vi "!GviewerMain.vi"() -> ()   [LabVIEW 2020, in "Sgraph_lib_V1.lvlib" / "Gviewer.lvclass"]
doc: "Main Graph Viewer.\nSeveral instances of this viewer can run simultaneously."
uses:
  Gviewer.lvclass
  controls/Typedef_Live.ctl
  Gserver/controls/Typedef_Gviewer-Query.ctl
  Gserver/controls/Typedef_QueryType.ctl
  controls/KeyPress.ctl
  <vilib>/event_ctls.llb/eventvkey.ctl
  Gviewer.lvclass/Gviewer.ctl
  FAMM/controls/FAMM_reply_datagram.ctl
  FAMM/controls/FAMM_reply_WAQdata.ctl
  FAMM/controls/FAMM_reply_EAQdata.ctl
  FAMM/controls/FAMM_reply_PAQdata.ctl
  controls/EditTagOneTag.ctl
  controls/Typedef_SelProperties.ctl
  controls/Typedef_LineType.ctl
  controls/Typedef_PresetSave.ctl
  controls/ToolBarAppearance.ctl
  controls/Typedef_Gserver-Replies.ctl
  controls/Typedef_ServerActions.ctl
  Common/controls/ToolTypeEnum.ctl
  Gserver/Gserver.lvclass
  FAMM/FAMM.lvclass
  Builds/Sgraph_lib_V1.lvlib
panel:
  out "TimeSpanText":string
  out "Key UP":T1 {"Time" format="%<%.3X>T"}
  out "Key DN":T1 {"Time" format="%<%.3X>T"}
  in  "StartupTagList":string[](array[string])
  in  "Gserver-Queue":refnum<queue>
  in  "GviewName":string="Gview-01"
  in  "Live":T3
  out "ToolBar":picture
  out "Graph":cluster{dbl[], "data":dbl[]}[](graph)
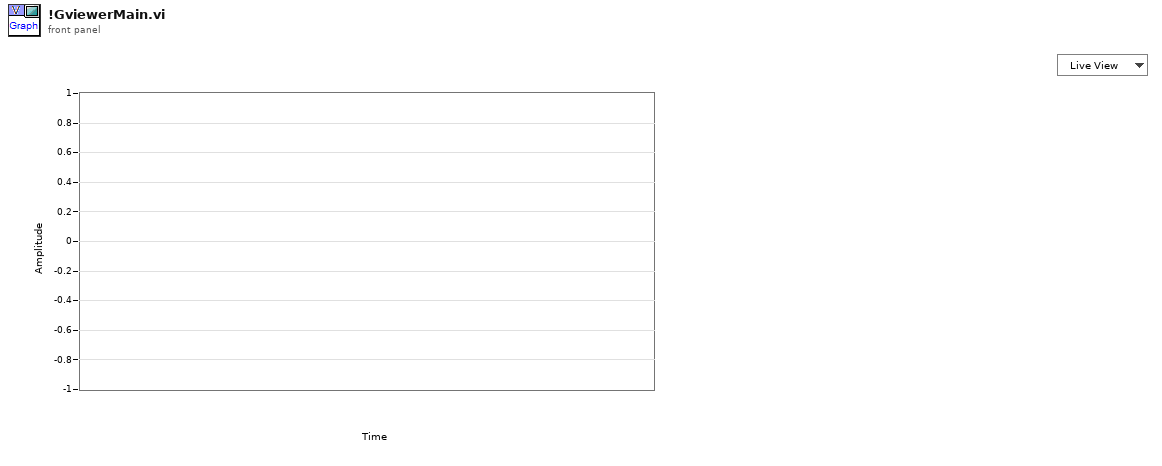
[diagram p1: front panel]
types:
  T1 = typedef "Sgraph_lib_V1.lvlib/Gviewer.lvclass/KeyPress.ctl" = cluster{"Char":i16, "VKey":T2, "Shift":bool, "Ctrl":bool, "Time":timestamp}
  T2 = typedef "eventvkey.ctl" = enum16{"ASCII", "Enter", "Return", "Shift", "Ctrl", "Alt", "Cmd", "Opt", "Caps", "NumLock", "Clear", "Break", "Up", "Down", "Left", "Right", "Insert", "Delete", "Home", "End", "PageUp", "PageDown", "Escape", "Help", "Pause", "ScrollLock", "F1", "F2", "F3", "F4", "F5", "F6", "F7", "F8", "F9", "F10", "F11", "F12", "F13", "F14", "F15", "F16", "F17", "F18", "F19", "F20", "F21", "F22", "F23", "F24", "Play", "VolumeUp", "VolumeDown", "Mute", "Two Byte Char"}
  T3 = typedef "Sgraph_lib_V1.lvlib/Gviewer.lvclass/Typedef_Live.ctl" = enum16{"Live View", "Freeze"}
  T4 = typedef "Sgraph_lib_V1.lvlib/FAMM.lvclass/FAMM_reply_datagram.ctl" = cluster{"GraphName":string, "Time-Start":timestamp, "Time-End":timestamp, "TimeSpan":dbl, "Live":T3, "WAQ_section":T5, "EAQ_section":T6, "PAQ_section":T7, "Layer":i32}
  T5 = typedef "Sgraph_lib_V1.lvlib/FAMM.lvclass/FAMM_reply_WAQdata.ctl" = cluster{"Boolean":bool}
  T6 = typedef "Sgraph_lib_V1.lvlib/FAMM.lvclass/FAMM_reply_EAQdata.ctl" = cluster{"Boolean":bool}
  T7 = typedef "Sgraph_lib_V1.lvlib/FAMM.lvclass/FAMM_reply_PAQdata.ctl" = cluster{"Tags":string[], "time stamp":timestamp[], "DataSection":cluster{"data":dbl[], "max":dbl[], "min":dbl[], "Status":u32[]}[]}
  T8 = typedef "Sgraph_lib_V1.lvlib/Gviewer.lvclass/EditTagOneTag.ctl" = cluster{"TAG":string, "min":dbl, "max":dbl, "Color":u32}
  T9 = typedef "Sgraph_lib_V1.lvlib/Gviewer.lvclass/Typedef_LineType.ctl" = enum16{"num_bare", "num_MinMax_Area", "num_MinMax_Lines", "num_MinMax_Forfor", "num_Max_Area", "num_Max_Line", "num_Max_Forfor", "num_Min_Area", "num_Min_Line", "num_Min_Fosfor", "Boolean_Line_01", "Boolean_Area_01", "Boolean_Fosfor_01", "Boolean_Line_TF", "Boolean_Area_TF", "Boolean_Fosfor_TF", "Boolean_OnOff_Line", "Boolean_OnOff_Area", "Boolean_OnOff_Fosfor", "Boolean_spare", "StringEvent_Line", "StringEvent_TimeLine"}
  T10 = typedef "Sgraph_lib_V1.lvlib/Gviewer.lvclass/Typedef_SelProperties.ctl" = cluster{"Color":u32, "LineType":T9, "max":dbl, "min":dbl}
  T11 = cluster{"EditTagsOpen":bool, "ExitRef":refnum<vi>}
  T12 = typedef "Sgraph_lib_V1.lvlib/Gviewer.lvclass/Typedef_PresetSave.ctl" = cluster{"Save time?":bool, "Presets":T8[], "PresetFilePath":path}
  T13 = typedef "Sgraph_lib_V1.lvlib/Gserver.lvclass/Typedef_QueryType.ctl" = enum16{"Subscribe", "DataRequest", "RequestAllTags", "RequestIniPath", "FAMMstarted", "SetClientOptions", "GviewerUpdate", "OpenNewGraph", "CloseClient", "CloseAllClients", "Close Gserver", "OpenMemoryMap", "MeMapDataRequest", "MeMapDataResponse"}
  T14 = typedef "Sgraph_lib_V1.lvlib/Gviewer.lvclass/ToolBarAppearance.ctl" = enum16{"Bare", "Native", "Gradient"}
  T15 = typedef "Sgraph_lib_V1.lvlib/Typedef_ServerActions.ctl" = enum16{"GraphUpdate", "SendAllTags", "SendIniPath", "SetGeneralOptions", "EditTagsOpen", "EditTagsPresetSave", "EditTagsPresetLoad", "EditTagsClose", "NewTagSelection", "ExitGraph"}
  T16 = typedef "Typedef_Gserver-Replies.ctl" = cluster{"ServerActions":T15, "data":variant, "Source":string, "Time Stamp":timestamp}
  T17 = typedef "Sgraph_lib_V1.lvlib/ToolTypeEnum.ctl" = enum16{"Esc button", "one", "HelpButton", "CursorViewButton", "four", "five", "six", "seven", "eight", "nine", "ten", "eleven", "twelve", "thirteen", "fourteen", "fifteen", "sixteen", "seventeen", "eighteen", "nineteen", "VerticalScroll", "VerticalMove", "TimeScroll", "TimeHandMove", "twentyfour", "twentyfive", "ZoomWindow drag", "ZoomHorDragging", "ZoomVerticalDrag", "twentynine", "LegendMovePoint", "LegendMoveDrag", "Thirtytwo", "ThirtyThree", "ThirtyFour", "ThirgyFive", "ThirtySix", "ThirtySeven", "ThirtyEight", "ThirtyNine", "AddYscalePoint", "AddYscalePlace", "AddYscaleMovePoint", "AddYscaleMoveDrag", "AddYscaleDeletePoint"}
  T18 = typedef "Sgraph_lib_V1.lvlib/Gviewer.lvclass/SettingsGeneral.ctl" = cluster{"MenuBar_active":bool, "ContextMenu_active":bool}
  T19 = typedef "LVPositionTypeDef.ctl" = cluster{"Left":i32, "Top":i32}
  T20 = typedef "LVPoint32TypeDef.ctl" = cluster{"Horizontal":i32, "Vertical":i32}
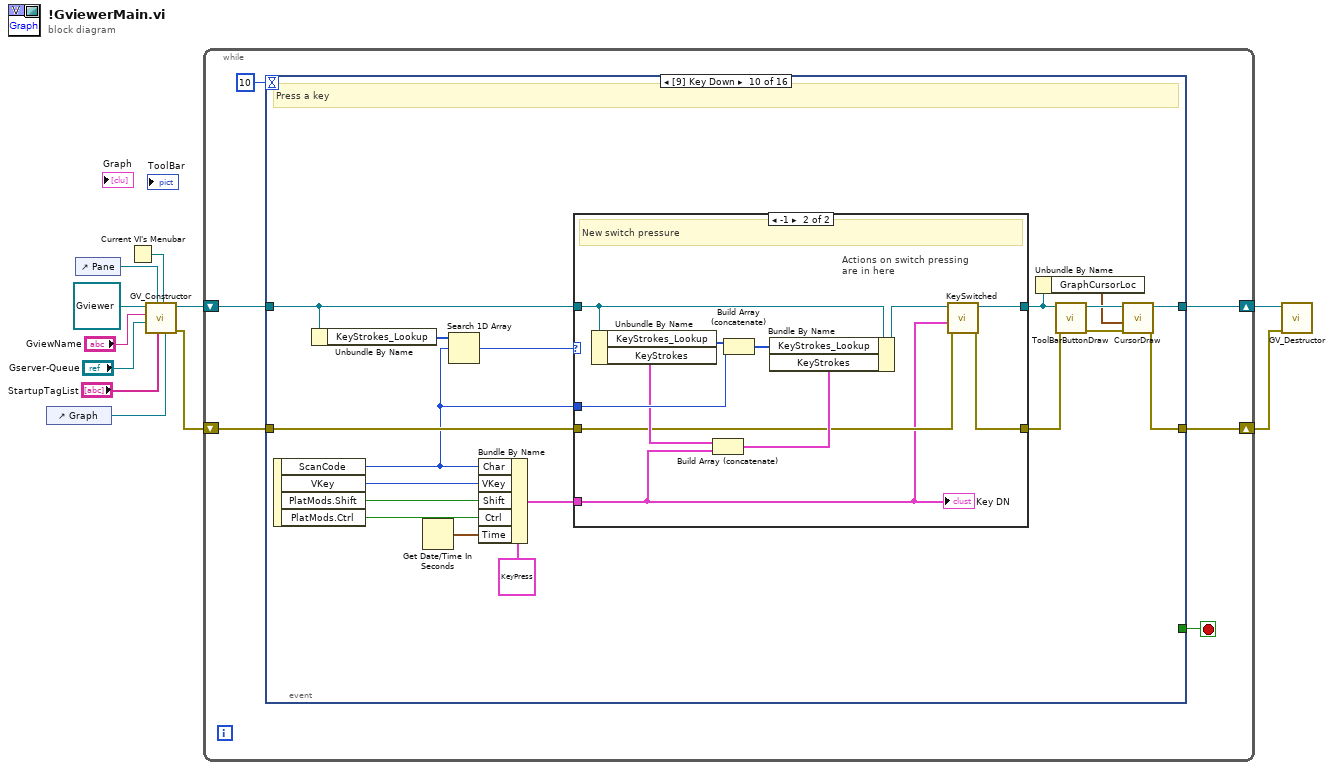
[diagram p0: block diagram]
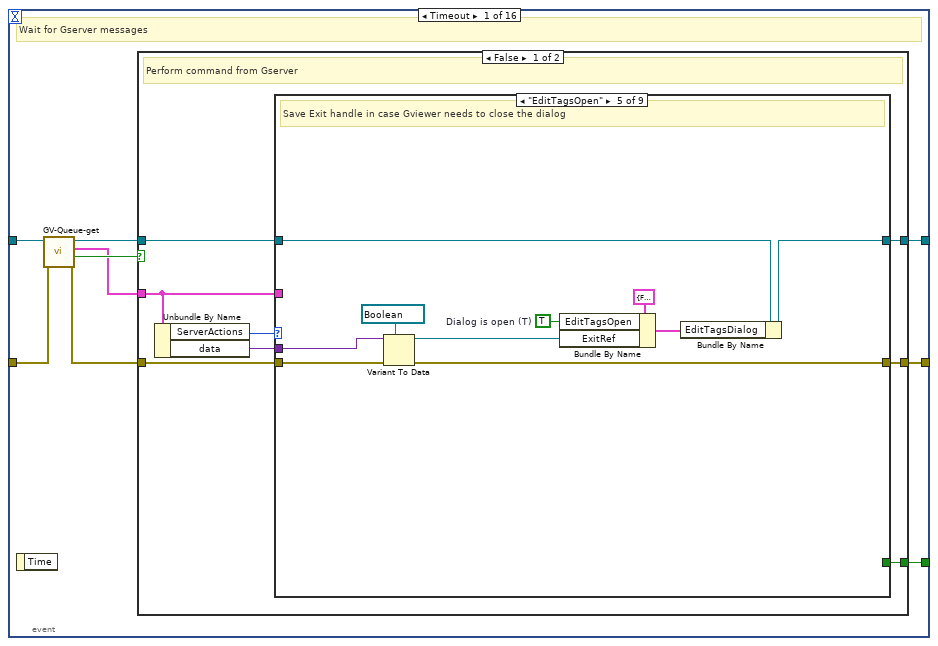
[diagram p2: hidden frame]
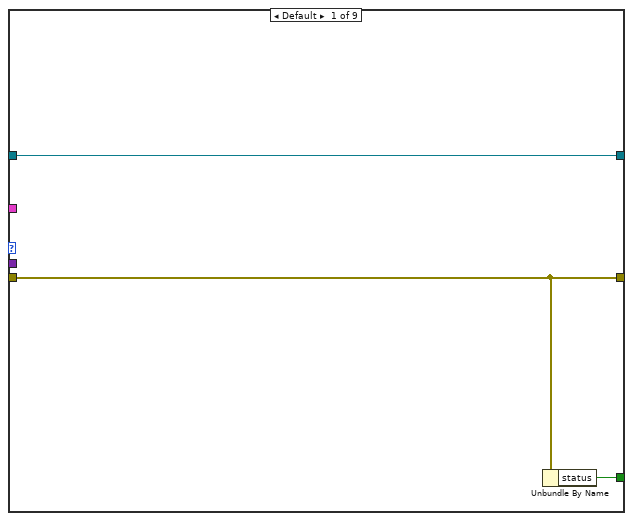
[diagram p3: hidden frame]
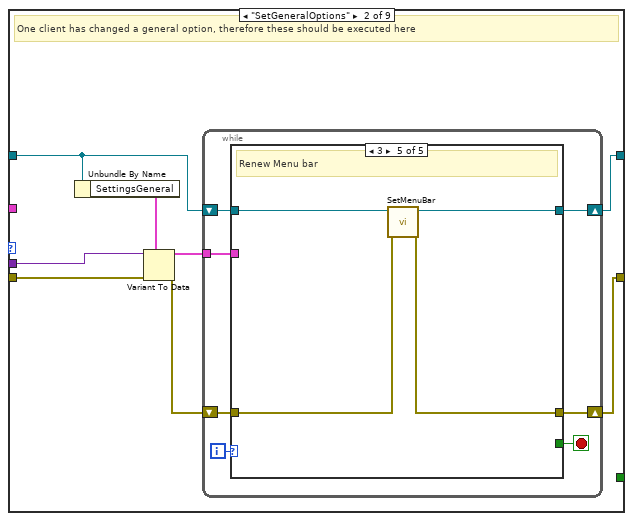
[diagram p4: hidden frame]
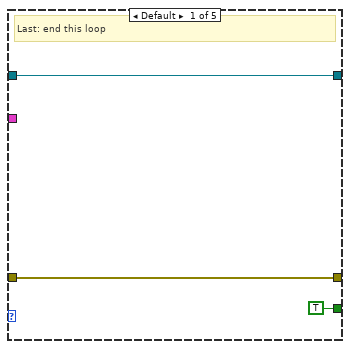
[diagram p5: hidden frame]
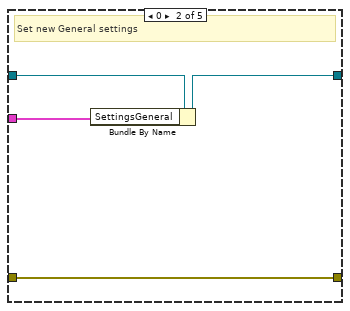
[diagram p6: hidden frame]
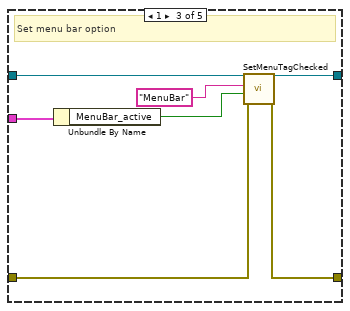
[diagram p7: hidden frame]
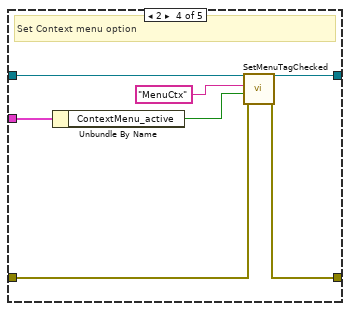
[diagram p8: hidden frame]
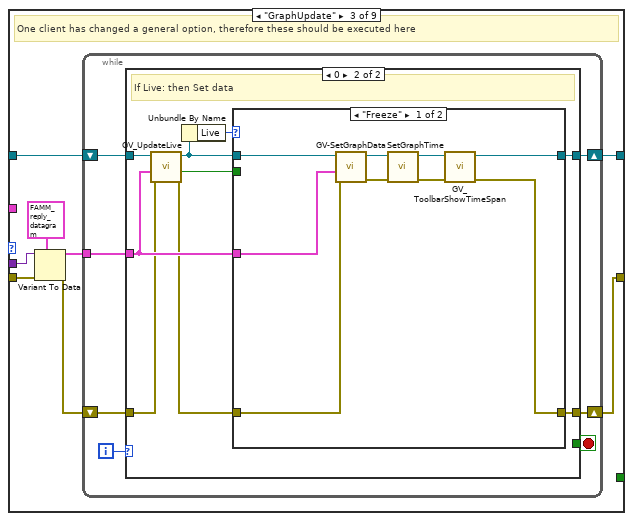
[diagram p9: hidden frame]
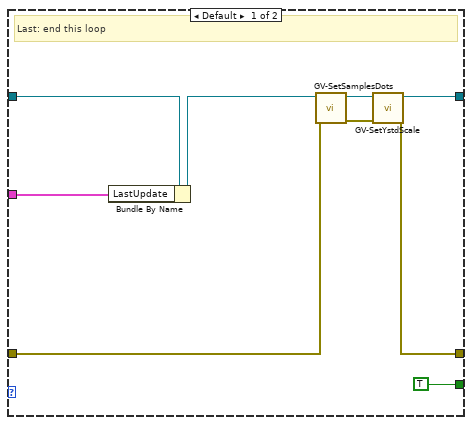
[diagram p10: hidden frame]
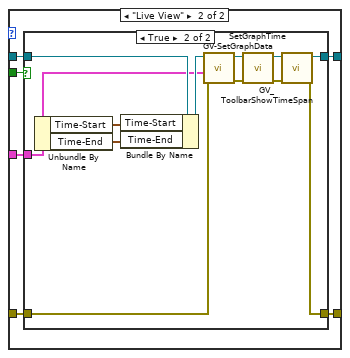
[diagram p11: hidden frame]
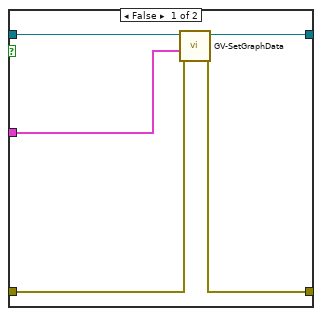
[diagram p12: hidden frame]
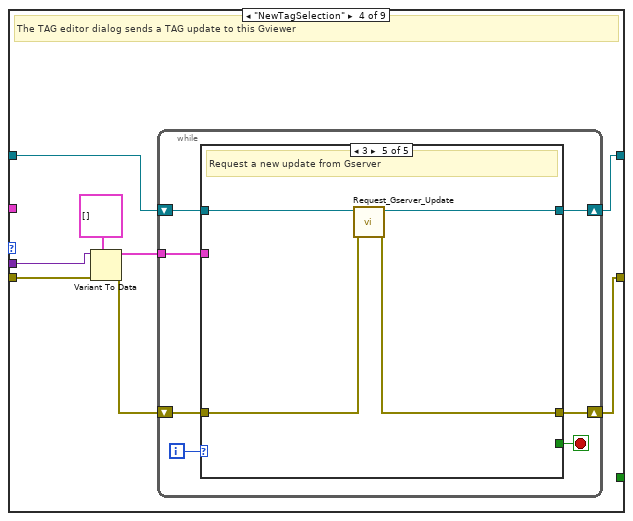
[diagram p13: hidden frame]
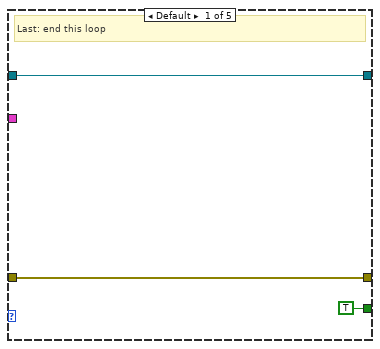
[diagram p14: hidden frame]
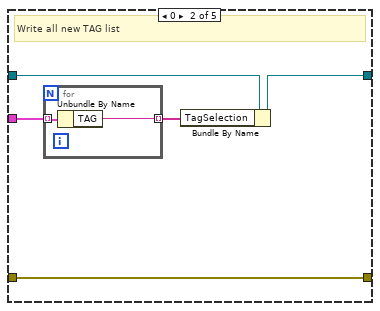
[diagram p15: hidden frame]
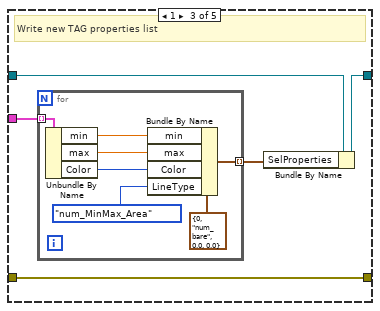
[diagram p16: hidden frame]
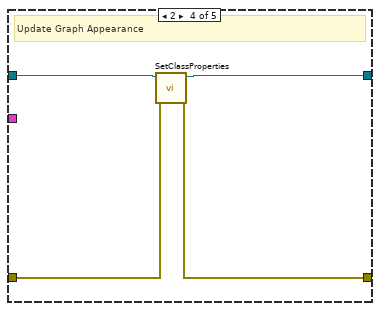
[diagram p17: hidden frame]
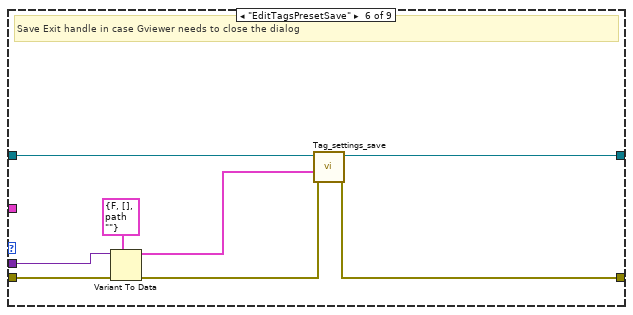
[diagram p18: hidden frame]
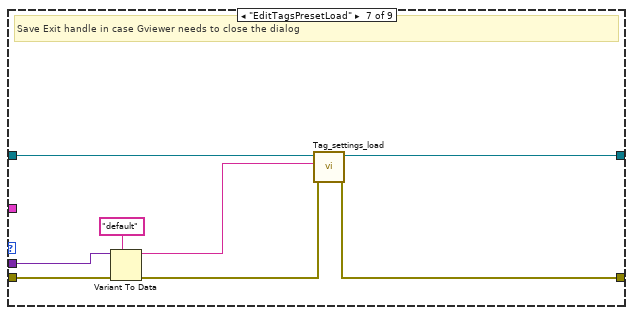
[diagram p19: hidden frame]
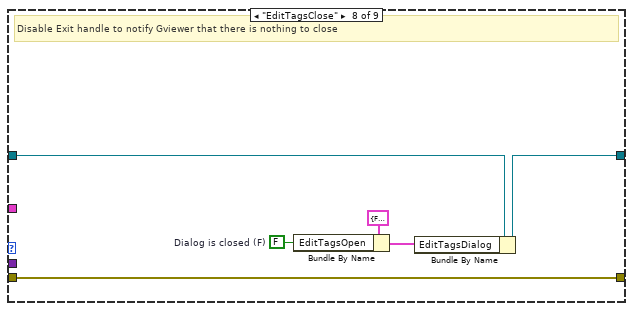
[diagram p20: hidden frame]
diagram:
  n1 = control-ref of="Graph"() -> (w2:refnum<vi>)
  n2 = control-ref of="Pane"() -> (w8:refnum<vi>)
  n3 = Current VI's Menubar() -> (w3:refnum<k9>)
  n4 = call "GV_Constructor.vi"("Graph-ref"=w2, "menu reference"=w3, "StartupTagList"="StartupTagList", "Pane"=w8, "Gserver-Queue"="Gserver-Queue", "GviewName"="GviewName", "Gviewer in"=refnum<class "Gviewer.lvclass"> refnum) -> ("error out"=w4:errorcluster, "Gviewer out"=w11:refnum<class "Gviewer.lvclass">)  [unwired: 3 in]
  n5 = while {
    shift-right: [w15] -> w1
    shift-left: w11 -> [w16]
    shift-right: [w13] -> w10
    shift-left: w4 -> [w14]
    stop <- w12 stop-if-true
    n6 = event shown="[9] Key Down" {
      selector: _ -> [_ _ _ _ _ _ _ _ _ _ _ _ _ _ _ _]
      dyn-events: _ -> [_ _ _ _ _ _ _ _ _ _ _ _ _ _ _ _]
      timeout: 10 -> [_ _ _ _ _ _ _ _ _ _ _ _ _ _ _ _]
      tunnel: w16 -> [w18 w245 w260 w600 w610 w620 w626 w633 w667 w679 w718 w740 w748 w757 w788 w792]
      tunnel: [w25 w239 w258 w593 w613 w621 w627 w631 w668 w674 w712 w741 w744 w750 w781 w791] -> w15
      tunnel: w14 -> [w21 w243 w259 w599 w615 w618 w624 w632 w665 w678 w717 w738 w747 w755 w779 w789]
      tunnel: [w26 w241 w257 w592 w611 w619 w625 w630 w666 w672 w709 w739 w742 w752 w780 w789] -> w13
      tunnel: [w24 _ _ _ _ _ _ _ _ _ _ _ _ _ _ _] -> w12
      event Timeout {
        # "Wait for Gserver messages"
        n7 = event-data() -> ()  [unwired: 1 in, 1 out]
        n8 = call "GV-Queue-get.vi"("error in (no error)"=w21, "Gviewer in"=w18) -> ("error out"=w20:errorcluster, "Time-out"=w23:bool, "Query"=w22:T16, "Gviewer out"=w19:refnum<class "Gviewer.lvclass">)  [unwired: 5 in, 1 out]
        n9 = case shown="False" w23 {
          tunnel: w22 -> [w28 _]
          tunnel: w19 -> [w33 w236]
          tunnel: w20 -> [w32 w234]
          tunnel: [w31 w235] -> w26
          tunnel: [w30 w233] -> w25
          tunnel: [w29 w237] -> w24
          frame False {
            # "Perform command from Gserver"
            n10 = Unbundle By Name(w28) -> ("ServerActions"=w34:T15, "data"=w27:variant)
            n11 = case shown="\"EditTagsOpen\"" w34 {
              tunnel: w33 -> [w37 w39 w80 w145 w192 w201 w211 w218 w225]
              tunnel: w32 -> [w35 w44 w84 w149 w194 w204 w212 w214 w222]
              tunnel: [w35 w40 w81 w146 w195 w198 w208 w214 w220] -> w31
              tunnel: [w37 w42 w83 w148 w193 w202 w210 w219 w225] -> w30
              tunnel: [w36 _ _ _ _ _ _ _ TRUE] -> w29
              tunnel: w28 -> [_ _ _ _ _ _ _ _ _]
              tunnel: w27 -> [_ w45 w85 w150 w197 w205 w213 _ _]
              frame Default {
                n12 = Unbundle By Name(w35) -> ("status"=w36:bool)
              }
              frame "SetGeneralOptions" {
                # "One client has changed a general option, therefore these should be executed here"
                n13 = Unbundle By Name(w39) -> ("SettingsGeneral"=w43:T18)
                n14 = Variant To Data(error in=w44, type=w43, Variant=w45) -> (data=w38:T18, error out=w41:errorcluster)
                n15 = while {
                  shift-right: [w47] -> w42
                  shift-left: w39 -> [w50]
                  shift-right: [w46] -> w40
                  shift-left: w41 -> [w49]
                  tunnel: w38 -> [w48]
                  i -> [w52]
                  stop <- w51 stop-if-true
                  n16 = case shown="3" w52 {
                    tunnel: [TRUE _ _ _ _] -> w51
                    tunnel: w50 -> [w53 w59 w61 w72 w77]
                    tunnel: w49 -> [w54 w56 w63 w68 w75]
                    tunnel: w48 -> [_ w58 w60 w70 _]
                    tunnel: [w53 w57 w65 w71 w76] -> w47
                    tunnel: [w54 w56 w62 w67 w74] -> w46
                    frame Default {
                      # "Last: end this loop"
                    }
                    frame 0 {
                      # "Set new General settings"
                      n17 = Bundle By Name(cluster=w59, "SettingsGeneral"=w58) -> (w57:refnum<class "Gviewer.lvclass">)
                    }
                    frame 1 {
                      # "Set menu bar option"
                      n18 = Unbundle By Name(w60) -> ("MenuBar_active"=w64:bool)
                      n19 = call "SetMenuTagChecked.vi"("error in (no error)"=w63, "Checked"=w64, "TAG"="MenuBar", "Gviewer in"=w61) -> ("error out"=w62:errorcluster, "Gviewer out"=w65:refnum<class "Gviewer.lvclass">)  [unwired: 6 in]
                    }
                    frame 2 {
                      # "Set Context menu option"
                      n20 = Unbundle By Name(w70) -> ("ContextMenu_active"=w69:bool)
                      n21 = call "SetMenuTagChecked.vi"("error in (no error)"=w68, "Checked"=w69, "TAG"="MenuCtx", "Gviewer in"=w72) -> ("error out"=w67:errorcluster, "Gviewer out"=w71:refnum<class "Gviewer.lvclass">)  [unwired: 6 in]
                    }
                    frame 3 {
                      # "Renew Menu bar"
                      n22 = call "SetMenuBar.vi"("error in (no error)"=w75, "Gviewer in"=w77) -> ("error out"=w74:errorcluster, "Gviewer out"=w76:refnum<class "Gviewer.lvclass">)  [unwired: 8 in]
                    }
                  }
                }
              }
              frame "GraphUpdate" {
                # "One client has changed a general option, therefore these should be executed here"
                n23 = Variant To Data(error in=w84, type=T4 {"GraphName"="", "Time-Start"=timestamp(0 s since 1904-01-01), "Time-End"=timestamp(0 s since 1904-01-01), "TimeSpan"=0.0, "Live"=enum."Live View", "WAQ_section"={"Boolean"=FALSE}, "EAQ_section"={"Boolean"=FALSE}, "PAQ_section"={"Tags"=[], "time stamp"=[], "DataSection"=[]}, "Layer"=0} ("GviewerUpdate"), Variant=w85) -> (data=w79:T4, error out=w82:errorcluster)
                n24 = while {
                  shift-right: [w87] -> w83
                  shift-left: w80 -> [w90]
                  shift-right: [w86] -> w81
                  shift-left: w82 -> [w89]
                  tunnel: w79 -> [w88]
                  i -> [w92]
                  stop <- w91 stop-if-true
                  n25 = case shown="0" w92 {
                    tunnel: [TRUE _] -> w91
                    tunnel: w90 -> [w97 w108]
                    tunnel: w89 -> [w93 w105]
                    tunnel: w88 -> [w98 w107]
                    tunnel: [w99 w110] -> w87
                    tunnel: [w100 w109] -> w86
                    frame Default {
                      # "Last: end this loop"
                      n26 = Bundle By Name(cluster=w97, "LastUpdate"=w98) -> (w96:refnum<class "Gviewer.lvclass">)
                      n27 = call "GV-SetSamplesDots.vi"("error in (no error)"=w93, "Gviewer in"=w96) -> ("error out"=w94:errorcluster, "Gviewer out"=w95:refnum<class "Gviewer.lvclass">)  [unwired: 8 in]
                      n28 = call "GV-SetYstdScale.vi"("error in (no error)"=w94, "Gviewer in"=w95) -> ("error out"=w100:errorcluster, "Gviewer out"=w99:refnum<class "Gviewer.lvclass">)  [unwired: 8 in]
                    }
                    frame 0 {
                      # "If Live: then Set data"
                      n29 = call "GV_UpdateLive.vi"("error in (no error)"=w105, "GviewerUpdate"=w107, "Gviewer in"=w108) -> ("error out"=w106:errorcluster, "RollTime?"=w102:bool, "Gviewer out"=w104:refnum<class "Gviewer.lvclass">)  [unwired: 6 in]
                      n30 = Unbundle By Name(w104) -> ("Live"=w103:T3)
                      n31 = case shown="\"Freeze\"" w103 {
                        tunnel: w104 -> [w119 w125]
                        tunnel: [w113 w124] -> w110
                        tunnel: w106 -> [w118 w123]
                        tunnel: [w111 w122] -> w109
                        tunnel: w107 -> [w117 w121]
                        tunnel: w102 -> [_ w120]
                        frame "Freeze" {
                          n32 = call "GV-SetGraphData.vi"("error in (no error)"=w118, "GviewerUpdate"=w117, "Gviewer in"=w119) -> ("error out"=w115:errorcluster, "Gviewer out"=w116:refnum<class "Gviewer.lvclass">)  [unwired: 7 in]
                          n33 = call "SetGraphTime.vi"("error in (no error)"=w115, "Gviewer in"=w116) -> ("error out"=w112:errorcluster, "Gviewer out"=w114:refnum<class "Gviewer.lvclass">)  [unwired: 8 in]
                          n34 = call "GV_ToolbarShowTimeSpan.vi"("error in (no error)"=w112, "Gviewer in"=w114) -> ("error out"=w111:errorcluster, "Gviewer out"=w113:refnum<class "Gviewer.lvclass">)  [unwired: 7 in, 1 out]
                        }
                        frame "Live View" {
                          n35 = case shown="True" w120 {
                            tunnel: w125 -> [w130 w138]
                            tunnel: [w129 w132] -> w124
                            tunnel: w123 -> [w128 w142]
                            tunnel: [w127 w131] -> w122
                            tunnel: w121 -> [w126 w137]
                            frame False {
                              n36 = call "GV-SetGraphData.vi"("error in (no error)"=w128, "GviewerUpdate"=w126, "Gviewer in"=w130) -> ("error out"=w127:errorcluster, "Gviewer out"=w129:refnum<class "Gviewer.lvclass">)  [unwired: 7 in]
                            }
                            frame True {
                              n37 = Unbundle By Name(w137) -> ("Time-Start"=w135:timestamp, "Time-End"=w136:timestamp)
                              n38 = Bundle By Name(cluster=w138, "Time-Start"=w135, "Time-End"=w136) -> (w139:refnum<class "Gviewer.lvclass">)
                              n39 = call "GV-SetGraphData.vi"("error in (no error)"=w142, "GviewerUpdate"=w137, "Gviewer in"=w139) -> ("error out"=w140:errorcluster, "Gviewer out"=w141:refnum<class "Gviewer.lvclass">)  [unwired: 7 in]
                              n40 = call "SetGraphTime.vi"("error in (no error)"=w140, "Gviewer in"=w141) -> ("error out"=w133:errorcluster, "Gviewer out"=w134:refnum<class "Gviewer.lvclass">)  [unwired: 8 in]
                              n41 = call "GV_ToolbarShowTimeSpan.vi"("error in (no error)"=w133, "Gviewer in"=w134) -> ("error out"=w131:errorcluster, "Gviewer out"=w132:refnum<class "Gviewer.lvclass">)  [unwired: 7 in, 1 out]
                            }
                          }
                        }
                      }
                    }
                  }
                }
              }
              frame "NewTagSelection" {
                # "The TAG editor dialog sends a TAG update to this Gviewer"
                n42 = Variant To Data(error in=w149, type=T8[] [] ("Presets"), Variant=w150) -> (data=w144:T8[], error out=w147:errorcluster)
                n43 = while {
                  shift-right: [w152] -> w148
                  shift-left: w145 -> [w155]
                  shift-right: [w151] -> w146
                  shift-left: w147 -> [w154]
                  tunnel: w144 -> [w153]
                  i -> [w157]
                  stop <- w156 stop-if-true
                  n44 = case shown="3" w157 {
                    tunnel: [TRUE _ _ _ _] -> w156
                    tunnel: w155 -> [w158 w164 w170 w183 w186]
                    tunnel: w154 -> [w159 w161 w172 w181 w184]
                    tunnel: w153 -> [_ w165 w169 _ _]
                    tunnel: [w158 w162 w171 w180 w187] -> w152
                    tunnel: [w159 w161 w172 w182 w185] -> w151
                    frame Default {
                      # "Last: end this loop"
                    }
                    frame 0 {
                      # "Write all new TAG list"
                      n45 = for {
                        tunnel: w165 -> [w167] mode=indexing
                        tunnel: [w166] -> w163 mode=indexing
                        n46 = Unbundle By Name(w167) -> ("TAG"=w166:string)
                      }
                      n47 = Bundle By Name(cluster=w164, "TagSelection"=w163) -> (w162:refnum<class "Gviewer.lvclass">)
                    }
                    frame 1 {
                      # "Write new TAG properties list"
                      n48 = for {
                        tunnel: w169 -> [w179] mode=indexing
                        tunnel: [w173] -> w168 mode=indexing
                        n49 = Unbundle By Name(w179) -> ("min"=w177:dbl, "max"=w176:dbl, "Color"=w175:u32)
                        n50 = Bundle By Name(cluster=T10 {"Color"=0, "LineType"=enum."num_bare", "max"=0.0, "min"=0.0} ("SelProperties"), "min"=w177, "max"=w176, "Color"=w175, "LineType"=Typedef_LineType."num_MinMax_Area") -> (w173:T10)
                      }
                      n51 = Bundle By Name(cluster=w170, "SelProperties"=w168) -> (w171:refnum<class "Gviewer.lvclass">)
                    }
                    frame 2 {
                      # "Update Graph Appearance"
                      n52 = call "SetClassProperties.vi"("error in (no error)"=w181, "Gviewer in"=w183) -> ("error out"=w182:errorcluster, "Gviewer out"=w180:refnum<class "Gviewer.lvclass">)  [unwired: 8 in]
                    }
                    frame 3 {
                      # "Request a new update from Gserver"
                      n53 = call "Request_Gserver_Update.vi"("error in (no error)"=w184, "Gviewer in"=w186) -> ("error out"=w185:errorcluster, "Gviewer out"=w187:refnum<class "Gviewer.lvclass">)  [unwired: 8 in]
                    }
                  }
                }
              }
              frame "EditTagsOpen" {
                w190 = TRUE  # Dialog is open (T)
                # "Save Exit handle in case Gviewer needs to close the dialog"
                n54 = Variant To Data(error in=w194, type=refnum<vi> refnum ("Exit_event"), Variant=w197) -> (data=w189:refnum<vi>, error out=w195:errorcluster)
                n55 = Bundle By Name(cluster=T11 {"EditTagsOpen"=FALSE, "ExitRef"=refnum} ("EditTagsDialog"), "EditTagsOpen"=w190, "ExitRef"=w189) -> (w188:T11)
                n56 = Bundle By Name(cluster=w192, "EditTagsDialog"=w188) -> (w193:refnum<class "Gviewer.lvclass">)
              }
              frame "EditTagsPresetSave" {
                # "Save Exit handle in case Gviewer needs to close the dialog"
                n57 = Variant To Data(error in=w204, type=T12 {"Save time?"=FALSE, "Presets"=[], "PresetFilePath"=path ""} ("PresetSave"), Variant=w205) -> (data=w200:T12, error out=w199:errorcluster)
                n58 = call "Tag_settings_save.vi"("error in (no error)"=w199, "PresetSave"=w200, "Gviewer in"=w201) -> ("error out"=w198:errorcluster, "Gviewer out"=w202:refnum<class "Gviewer.lvclass">)  [unwired: 7 in]
              }
              frame "EditTagsPresetLoad" {
                # "Save Exit handle in case Gviewer needs to close the dialog"
                n59 = Variant To Data(error in=w212, type="default", Variant=w213) -> (data=w206:string, error out=w209:errorcluster)
                n60 = call "Tag_settings_load.vi"("error in (no error)"=w209, "PresetName"=w206, "Gviewer in"=w211) -> ("error out"=w208:errorcluster, "Gviewer out"=w210:refnum<class "Gviewer.lvclass">)  [unwired: 7 in]
              }
              frame "EditTagsClose" {
                w216 = FALSE  # Dialog is closed (F)
                # "Disable Exit handle to notify Gviewer that there is nothing to close"
                n61 = Bundle By Name(cluster=T11 {"EditTagsOpen"=FALSE, "ExitRef"=refnum} ("EditTagsDialog"), "EditTagsOpen"=w216) -> (w215:T11)
                n62 = Bundle By Name(cluster=w218, "EditTagsDialog"=w215) -> (w219:refnum<class "Gviewer.lvclass">)
              }
              frame "ExitGraph" {
                # "Exit this Graph application (shutdown asked by Gserver)"
                n63 = Unbundle By Name(w225) -> ("EditTagsDialog"=w224:T11)
                n64 = Unbundle By Name(w224) -> ("ExitRef"=w221:refnum<vi>, "EditTagsOpen"=w223:bool)
                n65 = case "Close TAG edit dialog" shown="True" w223 {
                  selector: w223 -> [_ w229]
                  tunnel: w222 -> [w227 w231]
                  tunnel: w221 -> [_ w232]
                  tunnel: [w227 w230] -> w220
                  frame False {
                  }
                  frame True {
                    n66 = To Variant(anything=w229) -> (Variant=w228:variant)
                    n67 = property class="Bool"(reference=w232, error in=w231, "Val(Sgnl)"=w228) -> (error out=w230:errorcluster)  [unwired: 1 out]
                  }
                }
              }
            }
          }
          frame True {
            # "Receiving Queue time-out"
            n68 = call "GV-EventsProcessing.vi"("error in (no error)"=w234, "Gviewer in"=w236) -> ("error out"=w235:errorcluster, "Gviewer out"=w233:refnum<class "Gviewer.lvclass">)  [unwired: 8 in]
            n69 = Unbundle By Name(w235) -> ("status"=w237:bool)
          }
        }
      }
      event Shortcut Menu Activation? {
        # "Right mouse click menu selection"
        n70 = event-data() -> ("MenuRef"=w244:refnum<k9>)  [unwired: 1 in]
        n71 = Unbundle By Name(w245) -> ("Context_set"=w246:bool)
        n72 = case shown="False" w246 {
          selector: w246 -> [w252 _]
          tunnel: w245 -> [w249 w253]
          tunnel: w244 -> [w250 w255]
          tunnel: w243 -> [w247 w256]
          tunnel: [w247 w256] -> w240
          tunnel: [w248 w254] -> w242
          frame False {
            n73 = Not(x=w252) -> (.not. x?=w251:bool)
            n74 = Bundle By Name(cluster=w249, "Context_set"=w251, "Context-ref"=w250) -> (w248:refnum<class "Gviewer.lvclass">)
          }
          frame True {
            n75 = Bundle By Name(cluster=w253, "Context-ref"=w255) -> (w254:refnum<class "Gviewer.lvclass">)
          }
        }
        n76 = call "SetContextMenu.vi"("error in (no error)"=w240, "Gviewer in"=w242) -> ("error out"=w241:errorcluster, "Gviewer out"=w239:refnum<class "Gviewer.lvclass">)  [unwired: 8 in]
        n77 = event-data("Discard?"=FALSE) -> ()  [unwired: 1 in, 1 out]
      }
      event Menu Selection (User); Shortcut Menu Selection (User) {
        # "Menu bar action"
        n78 = event-data() -> ("ItemTag"=w261:string)  [unwired: 1 in]
        n79 = case shown="\"Yscale_add\"" w261 {
          selector: w261 -> [_ _ _ _ w312 _ w509 _ _ w574 _ w586]
          tunnel: w260 -> [w265 w270 w280 w294 w310 w492 w507 w518 w521 w569 w575 w587]
          tunnel: w259 -> [w264 w269 w274 w293 w309 w489 w510 w516 w535 w565 w582 w583]
          tunnel: [w266 w271 w276 w299 w307 w491 w512 w519 w521 w562 w576 w587] -> w258
          tunnel: [w263 w268 w275 w297 w305 w490 w511 w517 w536 w559 w582 w583] -> w257
          frame "Exit" {
            # "Send Exit command to Gserver (Gserver will then close this application)"
            n80 = call "SendDataToServer.vi"("error in (no error)"=w264, "Query_type"=Typedef_QueryType."CloseClient", "Gviewer in"=w265) -> ("error out"=w263:errorcluster, "Gviewer out"=w266:refnum<class "Gviewer.lvclass">)  [unwired: 7 in]
          }
          frame "ExitAll" {
            # "Send Exit command to Gserver (Gserver will then close this application)"
            n81 = call "SendDataToServer.vi"("error in (no error)"=w269, "Query_type"=Typedef_QueryType."CloseAllClients", "Gviewer in"=w270) -> ("error out"=w268:errorcluster, "Gviewer out"=w271:refnum<class "Gviewer.lvclass">)  [unwired: 7 in]
          }
          frame "MenuBar" {
            # "Options: Menu bar"
            n82 = Unbundle By Name(w280) -> ("SettingsGeneral"=w282:T18)
            n83 = Unbundle By Name(w282) -> ("MenuBar_active"=w283:bool, "ContextMenu_active"=w279:bool)
            n84 = case shown="True" w283 {
              selector: w283 -> [w286 w288]
              tunnel: [w285 w290] -> w281
              tunnel: w279 -> [w284 w289]
              tunnel: [w284 w287] -> w278
              frame False {
                n85 = Not(x=w286) -> (.not. x?=w285:bool)
              }
              frame True {
                # "Contect bar must be active\nif menu bar is set to OFF"
                n86 = Or(x=w288, y=w289) -> (x .or. y?=w287:bool)
                n87 = Not(x=w288) -> (.not. x?=w290:bool)
              }
            }
            n88 = Bundle By Name(cluster=w282, "MenuBar_active"=w281, "ContextMenu_active"=w278) -> (w272:T18)
            n89 = Bundle By Name(cluster=w280, "SettingsGeneral"=w272) -> (w277:refnum<class "Gviewer.lvclass">)
            n90 = call "SendDataToServer.vi"("error in (no error)"=w274, "data"=w272, "Query_type"=Typedef_QueryType."SetClientOptions", "Gviewer in"=w277) -> ("error out"=w275:errorcluster, "Gviewer out"=w276:refnum<class "Gviewer.lvclass">)  [unwired: 6 in]
          }
          frame "Legend" {
            # "Options: Legend on/off"
            n91 = call "GV_LegendVisible.vi"("error in (no error)"=w293, "Gviewer in"=w294) -> ("error out"=w291:errorcluster, "Visible?"=w292:bool, "Gviewer out"=w295:refnum<class "Gviewer.lvclass">)  [unwired: 7 in]
            n92 = call "SetMenuTagChecked.vi"("error in (no error)"=w291, "Checked"=w292, "TAG"="Legend", "Gviewer in"=w295) -> ("error out"=w298:errorcluster, "Gviewer out"=w300:refnum<class "Gviewer.lvclass">)  [unwired: 6 in]
            n93 = call "SetMenuBar.vi"("error in (no error)"=w298, "Gviewer in"=w300) -> ("error out"=w297:errorcluster, "Gviewer out"=w299:refnum<class "Gviewer.lvclass">)  [unwired: 8 in]
          }
          frame "T_000".."T_zzz" {
            # "Set Timeline"
            n94 = Get Date/Time In Seconds() -> (seconds since 1Jan1904=w311:timestamp)
            n95 = case shown="\"T_8hr\"" w312 {
              tunnel: w311 -> [_ _ _ _ _ _ _ w368 w381 w394 w407 _ _ _ _ _ _ _ _ _]
              tunnel: w310 -> [w314 w316 w324 w332 w340 w348 w356 w374 w387 w400 w413 w416 w424 w432 w440 w448 w456 w464 w472 w480]
              tunnel: w309 -> [w313 w322 w330 w338 w346 w354 w362 w371 w384 w397 w410 w422 w430 w438 w446 w454 w462 w470 w478 w486]
              tunnel: [w314 w318 w326 w334 w342 w350 w358 w375 w388 w401 w414 w418 w426 w434 w442 w450 w458 w466 w474 w482] -> w304
              tunnel: [w313 w322 w330 w338 w346 w354 w362 w369 w382 w395 w408 w422 w430 w438 w446 w454 w462 w470 w478 w486] -> w302
              frame Default {
                # "Not familiar.. Don't change"
              }
              frame "T_30sec" {
                w317 = 30.0  # 30 seconds
                # "Time span selected: 30 seconds"
                n96 = Unbundle By Name(w316) -> ("Time-End"=w315:timestamp)
                n97 = To Double Precision Float(number=w315) -> (double precision float=w321:dbl)
                n98 = Subtract(x=w321, y=w317) -> (x-y=w320:dbl)
                n99 = To Time Stamp(1:w320) -> (0:w319:timestamp)
                n100 = Bundle By Name(cluster=w316, "Time-Start"=w319, "TimeSpan(sec)"=w317) -> (w318:refnum<class "Gviewer.lvclass">)
              }
              frame "T_2min" {
                w325 = 120.0  # 2 minutes
                # "Time span selected: 2 minutes"
                n101 = Unbundle By Name(w324) -> ("Time-End"=w323:timestamp)
                n102 = To Double Precision Float(number=w323) -> (double precision float=w329:dbl)
                n103 = Subtract(x=w329, y=w325) -> (x-y=w328:dbl)
                n104 = To Time Stamp(1:w328) -> (0:w327:timestamp)
                n105 = Bundle By Name(cluster=w324, "Time-Start"=w327, "TimeSpan(sec)"=w325) -> (w326:refnum<class "Gviewer.lvclass">)
              }
              frame "T_10min" {
                w333 = 600.0  # 10 minutes
                # "Time span selected: 10 minutes"
                n106 = Unbundle By Name(w332) -> ("Time-End"=w331:timestamp)
                n107 = To Double Precision Float(number=w331) -> (double precision float=w337:dbl)
                n108 = Subtract(x=w337, y=w333) -> (x-y=w336:dbl)
                n109 = To Time Stamp(1:w336) -> (0:w335:timestamp)
                n110 = Bundle By Name(cluster=w332, "Time-Start"=w335, "TimeSpan(sec)"=w333) -> (w334:refnum<class "Gviewer.lvclass">)
              }
              frame "T_1hr" {
                w341 = 3600.0  # 60 minutes
                # "Time span selected: 1 hour"
                n111 = Unbundle By Name(w340) -> ("Time-End"=w339:timestamp)
                n112 = To Double Precision Float(number=w339) -> (double precision float=w345:dbl)
                n113 = Subtract(x=w345, y=w341) -> (x-y=w344:dbl)
                n114 = To Time Stamp(1:w344) -> (0:w343:timestamp)
                n115 = Bundle By Name(cluster=w340, "Time-Start"=w343, "TimeSpan(sec)"=w341) -> (w342:refnum<class "Gviewer.lvclass">)
              }
              frame "T_4hr" {
                w349 = 14400.0  # 4 hours
                # "Time span selected: 4 hours"
                n116 = Unbundle By Name(w348) -> ("Time-End"=w347:timestamp)
                n117 = To Double Precision Float(number=w347) -> (double precision float=w353:dbl)
                n118 = Subtract(x=w353, y=w349) -> (x-y=w352:dbl)
                n119 = To Time Stamp(1:w352) -> (0:w351:timestamp)
                n120 = Bundle By Name(cluster=w348, "Time-Start"=w351, "TimeSpan(sec)"=w349) -> (w350:refnum<class "Gviewer.lvclass">)
              }
              frame "T_8hr" {
                w357 = 28800.0  # 8 hours
                # "Time span selected: 4 hours"
                n121 = Unbundle By Name(w356) -> ("Time-End"=w355:timestamp)
                n122 = To Double Precision Float(number=w355) -> (double precision float=w361:dbl)
                n123 = Subtract(x=w361, y=w357) -> (x-y=w360:dbl)
                n124 = To Time Stamp(1:w360) -> (0:w359:timestamp)
                n125 = Bundle By Name(cluster=w356, "Time-Start"=w359, "TimeSpan(sec)"=w357) -> (w358:refnum<class "Gviewer.lvclass">)
              }
              frame "T_Today" {
                w373 = "%<%Y-%j>T" ("format string")
                # "Year + Day number"
                # "Time span selected: Since beginning of Today"
                n126 = Format Into String(format string=w373, error in=w371, w368) -> (resulting string=w372:string, error out=w370:errorcluster)  [unwired: 1 in]
                n127 = Scan From String(format string=w373, input string=w372, error in=w370) -> (error out=w369:errorcluster, output 1=w367:timestamp)  [unwired: 2 in, 2 out]
                n128 = To Double Precision Float(number=w368) -> (double precision float=w365:dbl)
                n129 = To Double Precision Float(number=w367) -> (double precision float=w364:dbl)
                n130 = Subtract(x=w365, y=w364) -> (x-y=w366:dbl)
                n131 = Bundle By Name(cluster=w374, "Live"=Typedef_Live."Live View", "Time-End"=w368, "Time-Start"=w367, "TimeSpan(sec)"=w366) -> (w375:refnum<class "Gviewer.lvclass">)
              }
              frame "T_month" {
                w386 = "%<%Y-%m>T" ("format string")
                # "Year + Month"
                # "Time span selected: Since beginning of this month"
                n132 = Format Into String(format string=w386, error in=w384, w381) -> (resulting string=w385:string, error out=w383:errorcluster)  [unwired: 1 in]
                n133 = Scan From String(format string=w386, input string=w385, error in=w383) -> (error out=w382:errorcluster, output 1=w380:timestamp)  [unwired: 2 in, 2 out]
                n134 = To Double Precision Float(number=w381) -> (double precision float=w378:dbl)
                n135 = To Double Precision Float(number=w380) -> (double precision float=w377:dbl)
                n136 = Subtract(x=w378, y=w377) -> (x-y=w379:dbl)
                n137 = Bundle By Name(cluster=w387, "Live"=Typedef_Live."Live View", "Time-End"=w381, "Time-Start"=w380, "TimeSpan(sec)"=w379) -> (w388:refnum<class "Gviewer.lvclass">)
              }
              frame "T_Year" {
                w399 = "%<%Y>T" ("format string")
                # "Time span selected: Since beginning of the Year"
                n138 = Format Into String(format string=w399, error in=w397, w394) -> (resulting string=w398:string, error out=w396:errorcluster)  [unwired: 1 in]
                n139 = Scan From String(format string=w399, input string=w398, error in=w396) -> (error out=w395:errorcluster, output 1=w393:timestamp)  [unwired: 2 in, 2 out]
                n140 = To Double Precision Float(number=w394) -> (double precision float=w391:dbl)
                n141 = To Double Precision Float(number=w393) -> (double precision float=w390:dbl)
                n142 = Subtract(x=w391, y=w390) -> (x-y=w392:dbl)
                n143 = Bundle By Name(cluster=w400, "Live"=Typedef_Live."Live View", "Time-End"=w394, "Time-Start"=w393, "TimeSpan(sec)"=w392) -> (w401:refnum<class "Gviewer.lvclass">)
              }
              frame "T_Week" {
                w412 = "%<%Y-%W>T" ("format string")
                # "Year + Week number"
                # "Time span selected: since beginning of this week"
                n144 = Format Into String(format string=w412, error in=w410, w407) -> (resulting string=w411:string, error out=w409:errorcluster)  [unwired: 1 in]
                n145 = Scan From String(format string=w412, input string=w411, error in=w409) -> (error out=w408:errorcluster, output 1=w406:timestamp)  [unwired: 2 in, 2 out]
                n146 = To Double Precision Float(number=w407) -> (double precision float=w404:dbl)
                n147 = To Double Precision Float(number=w406) -> (double precision float=w403:dbl)
                n148 = Subtract(x=w404, y=w403) -> (x-y=w405:dbl)
                n149 = Bundle By Name(cluster=w413, "Live"=Typedef_Live."Live View", "Time-End"=w407, "Time-Start"=w406, "TimeSpan(sec)"=w405) -> (w414:refnum<class "Gviewer.lvclass">)
              }
              frame "T_1day" {
                w417 = 86400.0  # 1 day
                # "Time span selected: 1 day"
                n150 = Unbundle By Name(w416) -> ("Time-End"=w415:timestamp)
                n151 = To Double Precision Float(number=w415) -> (double precision float=w421:dbl)
                n152 = Subtract(x=w421, y=w417) -> (x-y=w420:dbl)
                n153 = To Time Stamp(1:w420) -> (0:w419:timestamp)
                n154 = Bundle By Name(cluster=w416, "Time-Start"=w419, "TimeSpan(sec)"=w417) -> (w418:refnum<class "Gviewer.lvclass">)
              }
              frame "T_2days" {
                w425 = 172800.0  # 2 days
                # "Time span selected: 2 days"
                n155 = Unbundle By Name(w424) -> ("Time-End"=w423:timestamp)
                n156 = To Double Precision Float(number=w423) -> (double precision float=w429:dbl)
                n157 = Subtract(x=w429, y=w425) -> (x-y=w428:dbl)
                n158 = To Time Stamp(1:w428) -> (0:w427:timestamp)
                n159 = Bundle By Name(cluster=w424, "Time-Start"=w427, "TimeSpan(sec)"=w425) -> (w426:refnum<class "Gviewer.lvclass">)
              }
              frame "T_5days" {
                w433 = 432000.0  # 5 days
                # "Time span selected: 5 days"
                n160 = Unbundle By Name(w432) -> ("Time-End"=w431:timestamp)
                n161 = To Double Precision Float(number=w431) -> (double precision float=w437:dbl)
                n162 = Subtract(x=w437, y=w433) -> (x-y=w436:dbl)
                n163 = To Time Stamp(1:w436) -> (0:w435:timestamp)
                n164 = Bundle By Name(cluster=w432, "Time-Start"=w435, "TimeSpan(sec)"=w433) -> (w434:refnum<class "Gviewer.lvclass">)
              }
              frame "T_1wk" {
                w441 = 604800.0  # 7 days
                # "Time span selected: 1 week"
                n165 = Unbundle By Name(w440) -> ("Time-End"=w439:timestamp)
                n166 = To Double Precision Float(number=w439) -> (double precision float=w445:dbl)
                n167 = Subtract(x=w445, y=w441) -> (x-y=w444:dbl)
                n168 = To Time Stamp(1:w444) -> (0:w443:timestamp)
                n169 = Bundle By Name(cluster=w440, "Time-Start"=w443, "TimeSpan(sec)"=w441) -> (w442:refnum<class "Gviewer.lvclass">)
              }
              frame "T_2wks" {
                w449 = 1209600.0  # 14 days
                # "Time span selected: 2 weeks"
                n170 = Unbundle By Name(w448) -> ("Time-End"=w447:timestamp)
                n171 = To Double Precision Float(number=w447) -> (double precision float=w453:dbl)
                n172 = Subtract(x=w453, y=w449) -> (x-y=w452:dbl)
                n173 = To Time Stamp(1:w452) -> (0:w451:timestamp)
                n174 = Bundle By Name(cluster=w448, "Time-Start"=w451, "TimeSpan(sec)"=w449) -> (w450:refnum<class "Gviewer.lvclass">)
              }
              frame "T_1month" {
                w457 = 2678400.0  # 31 days
                # "Time span selected: one month"
                n175 = Unbundle By Name(w456) -> ("Time-End"=w455:timestamp)
                n176 = To Double Precision Float(number=w455) -> (double precision float=w461:dbl)
                n177 = Subtract(x=w461, y=w457) -> (x-y=w460:dbl)
                n178 = To Time Stamp(1:w460) -> (0:w459:timestamp)
                n179 = Bundle By Name(cluster=w456, "Time-Start"=w459, "TimeSpan(sec)"=w457) -> (w458:refnum<class "Gviewer.lvclass">)
              }
              frame "T_3months" {
                w465 = 7948800.0  # 92 days
                # "Time span selected: 1/4 Year"
                n180 = Unbundle By Name(w464) -> ("Time-End"=w463:timestamp)
                n181 = To Double Precision Float(number=w463) -> (double precision float=w469:dbl)
                n182 = Subtract(x=w469, y=w465) -> (x-y=w468:dbl)
                n183 = To Time Stamp(1:w468) -> (0:w467:timestamp)
                n184 = Bundle By Name(cluster=w464, "Time-Start"=w467, "TimeSpan(sec)"=w465) -> (w466:refnum<class "Gviewer.lvclass">)
              }
              frame "T_6months" {
                w473 = 15811200.0  # 183 days
                # "Time span selected: 1/2 Year"
                n185 = Unbundle By Name(w472) -> ("Time-End"=w471:timestamp)
                n186 = To Double Precision Float(number=w471) -> (double precision float=w477:dbl)
                n187 = Subtract(x=w477, y=w473) -> (x-y=w476:dbl)
                n188 = To Time Stamp(1:w476) -> (0:w475:timestamp)
                n189 = Bundle By Name(cluster=w472, "Time-Start"=w475, "TimeSpan(sec)"=w473) -> (w474:refnum<class "Gviewer.lvclass">)
              }
              frame "T_1year" {
                w481 = 31536000.0  # 365 days
                # "Time span selected: one Year"
                n190 = Unbundle By Name(w480) -> ("Time-End"=w479:timestamp)
                n191 = To Double Precision Float(number=w479) -> (double precision float=w485:dbl)
                n192 = Subtract(x=w485, y=w481) -> (x-y=w484:dbl)
                n193 = To Time Stamp(1:w484) -> (0:w483:timestamp)
                n194 = Bundle By Name(cluster=w480, "Time-Start"=w483, "TimeSpan(sec)"=w481) -> (w482:refnum<class "Gviewer.lvclass">)
              }
            }
            n195 = call "Request_Gserver_Update.vi"("error in (no error)"=w302, "Gviewer in"=w304) -> ("error out"=w301:errorcluster, "Gviewer out"=w303:refnum<class "Gviewer.lvclass">)  [unwired: 8 in]
            n196 = call "SetGraphTime.vi"("error in (no error)"=w301, "Gviewer in"=w303) -> ("error out"=w306:errorcluster, "Gviewer out"=w308:refnum<class "Gviewer.lvclass">)  [unwired: 8 in]
            n197 = call "GV_DrawLiveBox.vi"("error in (no error)"=w306, "Gviewer in"=w308) -> ("error out"=w305:errorcluster, "Gviewer out"=w307:refnum<class "Gviewer.lvclass">)  [unwired: 8 in]
          }
          frame "MenuCtx" {
            # "Options: Context menu"
            n198 = Unbundle By Name(w492) -> ("SettingsGeneral"=w497:T18)
            n199 = Unbundle By Name(w497) -> ("ContextMenu_active"=w498:bool, "MenuBar_active"=w495:bool)
            n200 = case shown="True" w498 {
              selector: w498 -> [w501 w503]
              tunnel: [w500 w505] -> w496
              tunnel: w495 -> [w499 w504]
              tunnel: [w499 w502] -> w494
              frame False {
                n201 = Not(x=w501) -> (.not. x?=w500:bool)
              }
              frame True {
                # "menu bar must be active\nif context menu is set to OFF"
                n202 = Or(x=w503, y=w504) -> (x .or. y?=w502:bool)
                n203 = Not(x=w503) -> (.not. x?=w505:bool)
              }
            }
            n204 = Bundle By Name(cluster=w497, "ContextMenu_active"=w496, "MenuBar_active"=w494) -> (w488:T18)
            n205 = Bundle By Name(cluster=w492, "SettingsGeneral"=w488) -> (w487:refnum<class "Gviewer.lvclass">)
            n206 = call "SendDataToServer.vi"("error in (no error)"=w489, "data"=w488, "Query_type"=Typedef_QueryType."SetClientOptions", "Gviewer in"=w487) -> ("error out"=w490:errorcluster, "Gviewer out"=w491:refnum<class "Gviewer.lvclass">)  [unwired: 6 in]
          }
          frame "ToolBare", "ToolGradient", "ToolNative" {
            # "Toolbar appearance layout change"
            n207 = case shown="\"ToolGradient\"" w509 {
              tunnel: [ToolBarAppearance."Native" ("ToolBarAppearance") ToolBarAppearance."Bare" ("ToolBarAppearance") ToolBarAppearance."Gradient" ("ToolBarAppearance")] -> w506
              frame Default {
              }
              frame "ToolBare" {
              }
              frame "ToolGradient" {
              }
            }
            n208 = Bundle By Name(cluster=w507, "ToolBarAppearance"=w506) -> (w508:refnum<class "Gviewer.lvclass">)
            n209 = call "GV_SetToolbar.vi"("error in (no error)"=w510, "Gviewer in"=w508) -> ("error out"=w511:errorcluster, "Gviewer out"=w512:refnum<class "Gviewer.lvclass">)  [unwired: 8 in]
          }
          frame "Pres_edit" {
            # "Open Preset Dialog"
            n210 = call "GV-StartPreset.vi"("error in (no error)"=w516, "Gviewer in"=w518) -> ("error out"=w517:errorcluster, "Gviewer out"=w519:refnum<class "Gviewer.lvclass">)  [unwired: 8 in]
          }
          frame "Pres_save" {
            # "Save current Preset setting"
            n211 = Unbundle By Name(w521) -> ("TagSelection"=w530:string[], "SelProperties"=w529:T10[])
            n212 = Unbundle By Name(w521) -> ("SettingsName"=w520:string)
            n213 = Unbundle By Name(w521) -> ("Settings_path"=w527:path)
            n214 = disable-structure shown="Enabled" {
              disable-tunnel: w527 -> [w548 w549]
              disable-tunnel: path "Presets" ("name or relative path") -> [w546 w551]
              disable-tunnel: [w545 w550] -> w523
              frame Enabled {
                # "One general presets path for all Graphs"
                n215 = Strip Path(path=w548) -> (stripped path=w547:path)  [unwired: 1 out]
                n216 = Build Path(base path=w547, name or relative path=w546) -> (appended path=w545:path)
              }
              frame Disabled {
                # "Specific settings per Graph instance"
                n217 = Build Path(base path=w549, name or relative path=w551) -> (appended path=w550:path)
              }
            }
            n218 = for {
              tunnel: w530 -> [w557] mode=indexing
              tunnel: w529 -> [w556] mode=indexing
              tunnel: [w552] -> w528 mode=indexing
              n219 = Unbundle By Name(w556) -> ("min"=w555:dbl, "max"=w554:dbl, "Color"=w553:u32)
              n220 = Bundle By Name(cluster=T8 {"TAG"="", "min"=0.0, "max"=0.0, "Color"=0} ("Selected-Tag"), "TAG"=w557, "min"=w555, "max"=w554, "Color"=w553) -> (w552:T8)
            }
            n221 = Unbundle By Name(w521) -> ("Live"=w532:T3)
            n222 = Equal?(x=Typedef_Live."Freeze" ("y"), y=w532) -> (x = y?=w533:bool)
            n223 = Concatenate Strings(w520, ".sgp" ("string")) -> (w525:string)
            n224 = Build Path(base path=w523, name or relative path=w525) -> (appended path=w522:path)
            n225 = Bundle By Name(cluster=T12 {"Save time?"=FALSE, "Presets"=[], "PresetFilePath"=path ""} ("PresetSave"), "Save time?"=w533, "Presets"=w528, "PresetFilePath"=w522) -> (w537:T12)
            n226 = Get Date/Time In Seconds() -> (seconds since 1Jan1904=w544:timestamp)
            n227 = To Variant(anything=w537) -> (Variant=w538:variant)
            n228 = Bundle By Name(cluster=T16 {"ServerActions"=enum."GraphUpdate", "data"=variant, "Source"="", "Time Stamp"=timestamp(0 s since 1904-01-01)} ("element"), "data"=w538, "ServerActions"=Typedef_ServerActions."EditTagsPresetSave", "Source"="Edit TAGs dialog", "Time Stamp"=w544) -> (w543:T16)
            n229 = Unbundle By Name(w521) -> ("GViewer-Queue"=w534:refnum<queue>)
            n230 = Enqueue Element(queue=w534, element=w543, error in (no error)=w535) -> (error out=w536:errorcluster)  [unwired: 1 in, 2 out]
          }
          frame "preset_0000".."preset_9999" {
            n231 = Unbundle By Name(w569) -> ("PresetsAvailable"=w571:string[])
            n232 = Match Pattern(string=w574, regular expression="preset_") -> (after substring=w572:string)  [unwired: 1 in, 3 out]
            n233 = Decimal String To Number(string=w572) -> (number=w570:i32)  [unwired: 2 in, 1 out]
            n234 = Index Array(array=w571, index=w570) -> (element=w568:string)
            n235 = call "Tag_settings_load.vi"("error in (no error)"=w565, "PresetName"=w568, "Gviewer in"=w569) -> ("error out"=w567:errorcluster, "Gviewer out"=w566:refnum<class "Gviewer.lvclass">)  [unwired: 7 in]
            n236 = call "SetMenuBar.vi"("error in (no error)"=w567, "Gviewer in"=w566) -> ("error out"=w560:errorcluster, "Gviewer out"=w563:refnum<class "Gviewer.lvclass">)  [unwired: 8 in]
            n237 = call "SetClassProperties.vi"("error in (no error)"=w560, "Gviewer in"=w563) -> ("error out"=w561:errorcluster, "Gviewer out"=w564:refnum<class "Gviewer.lvclass">)  [unwired: 8 in]
            n238 = call "Request_Gserver_Update.vi"("error in (no error)"=w561, "Gviewer in"=w564) -> ("error out"=w559:errorcluster, "Gviewer out"=w562:refnum<class "Gviewer.lvclass">)  [unwired: 8 in]
          }
          frame "Yscale_add" {
            # "Add an Y-axis to the graph"
            n239 = Unbundle By Name(w575) -> ("PlotSelected"=w581:i32)
            n240 = Greater Or Equal To 0?(x=w581) -> (x >= 0?=w580:bool)
            n241 = Select(t=ToolTypeEnum."AddYscalePlace" ("Enum"), s=w580, f=ToolTypeEnum."AddYscalePoint" ("Enum")) -> (s? t:f=w577:T17)
            n242 = Bundle By Name(cluster=w575, "ToolButtonSelected"=w577) -> (w576:refnum<class "Gviewer.lvclass">)
          }
          frame Default {
            n243 = Concatenate Strings("Menu item not implemented:\n", w586) -> (w585:string)
            n244 = One Button Dialog(message=w585) -> ()  [unwired: 1 in, 1 out]
          }
        }
        n245 = disable-structure shown="Disabled" {
          frame Disabled {
            (unwired) ToolTypeEnum."VerticalMove" ("Enum")
          }
          frame Enabled {
          }
        }
      }
      event Pane Size {
        # "Rearange all objects to Pane size"
        n246 = event-data() -> ()  [unwired: 1 in, 3 out]
        n247 = call "GV_SetToolbar.vi"("error in (no error)"=w599, "Gviewer in"=w600) -> ("error out"=w597:errorcluster, "Gviewer out"=w598:refnum<class "Gviewer.lvclass">)  [unwired: 8 in]
        n248 = call "GV_SetGraph.vi"("error in (no error)"=w597, "Gviewer in"=w598) -> ("error out"=w595:errorcluster, "Gviewer out"=w596:refnum<class "Gviewer.lvclass">)  [unwired: 8 in]
        n249 = call "GV_DrawLiveBox.vi"("error in (no error)"=w595, "Gviewer in"=w596) -> ("error out"=w589:errorcluster, "Gviewer out"=w591:refnum<class "Gviewer.lvclass">)  [unwired: 8 in]
        n250 = call "GV_timedToolButtonsUpdate.vi"("error in (no error)"=w589, "Gviewer in"=w591) -> ("error out"=w588:errorcluster, "Gviewer out"=w590:refnum<class "Gviewer.lvclass">)  [unwired: 8 in]
        n251 = Unbundle By Name(w590) -> ("Visible"=w594:bool)
        n252 = case shown="True" w594 {
          tunnel: w590 -> [w602 w603]
          tunnel: [w602 w604] -> w593
          tunnel: w588 -> [w601 w605]
          tunnel: [w601 w606] -> w592
          frame False {
          }
          frame True {
            n253 = Unbundle By Name(w603) -> ("Graph-ref"=w608:refnum<vi>)
            n254 = property class="XYGraph (strict)"(reference=w608, error in=w605) -> (error out=w606:errorcluster, "LegPos"=w607:T19)  [unwired: 1 out]
            n255 = Bundle By Name(cluster=w603, "Position"=w607) -> (w604:refnum<class "Gviewer.lvclass">)
          }
        }
      }
      event "Graph": Mouse Move {
        # "Draw cursor info when mouse is moved"
        n256 = event-data() -> ("Coords"=w609:T20)  [unwired: 1 in]
        n257 = call "CursorDraw.vi"("error in (no error)"=w615, "Coords"=w609, "Gviewer in"=w610) -> ("error out"=w612:errorcluster, "Gviewer out"=w614:refnum<class "Gviewer.lvclass">)  [unwired: 7 in]
        n258 = call "GV_timedToolButtonsUpdate.vi"("error in (no error)"=w612, "Gviewer in"=w614) -> ("error out"=w611:errorcluster, "Gviewer out"=w613:refnum<class "Gviewer.lvclass">)  [unwired: 8 in]
      }
      event "Graph": Mouse Down {
        # "Click on a mouse button when on the graph"
        n259 = event-data() -> ("Button"=w616:u16, "Coords"=w617:T20)  [unwired: 1 in]
        n260 = call "GV-MouseDown.vi"("error in (no error)"=w618, "Coords"=w617, "Button"=w616, "Gviewer in"=w620) -> ("error out"=w619:errorcluster, "Gviewer out"=w621:refnum<class "Gviewer.lvclass">)  [unwired: 6 in]
      }
      event "Graph": Mouse Up {
        # "Release mouse while hovering over graph"
        n261 = event-data() -> ("Coords"=w623:T20)  [unwired: 1 in]
        n262 = call "GV-MouseUP.vi"("MouseLeave?"=FALSE, "error in (no error)"=w624, "Coords"=w623, "Gviewer in"=w626) -> ("error out"=w625:errorcluster, "Gviewer out"=w627:refnum<class "Gviewer.lvclass">)  [unwired: 6 in]
      }
      event "Graph": Mouse Wheel {
        # "Mouse scroll zoom functions"
        n263 = event-data() -> ("Coords"=w628:T20, "Delta"=w629:i32)  [unwired: 1 in]
        n264 = Unbundle By Name(w633) -> ("ToolButtonSelected"=w634:i32)
        n265 = case shown="20" w634 {
          tunnel: w633 -> [w636 w648 w663]
          tunnel: w632 -> [w635 w647 w660]
          tunnel: [w636 w639 w651] -> w631
          tunnel: [w635 w638 w650] -> w630
          tunnel: w629 -> [_ w646 w661]
          tunnel: w628 -> [_ w645 w662]
          frame Default {
            # "Not identified"
          }
          frame 20 {
            w637 = FALSE  # F = When scrolling is done
            # "Vertical Scroll zoom"
            n266 = call "Scroll-Vzoom.vi"("error in (no error)"=w647, "Scroll value"=w646, "Coords"=w645, "Gviewer in"=w648) -> ("error out"=w644:errorcluster, "Gviewer out"=w643:refnum<class "Gviewer.lvclass">)  [unwired: 6 in]
            n267 = Unbundle By Name(w643) -> ("LastUpdate"=w642:T4)
            n268 = call "GV-SetGraphData.vi"("error in (no error)"=w644, "GviewerUpdate"=w642, "Gviewer in"=w643) -> ("error out"=w640:errorcluster, "Gviewer out"=w641:refnum<class "Gviewer.lvclass">)  [unwired: 7 in]
            n269 = call "GV_StoreNewZoomValue.vi"("Immediate"=w637, "error in (no error)"=w640, "Gviewer in"=w641) -> ("error out"=w638:errorcluster, "Gviewer out"=w639:refnum<class "Gviewer.lvclass">)  [unwired: 7 in]
          }
          frame 22 {
            w649 = FALSE  # F = when scrolling is done
            # "Time zoom"
            n270 = call "Scroll-Hzoom.vi"("error in (no error)"=w660, "Scroll value"=w661, "Coords"=w662, "Gviewer in"=w663) -> ("error out"=w654:errorcluster, "Gviewer out"=w657:refnum<class "Gviewer.lvclass">)  [unwired: 6 in]
            n271 = call "Request_Gserver_Update.vi"("error in (no error)"=w654, "Gviewer in"=w657) -> ("error out"=w658:errorcluster, "Gviewer out"=w659:refnum<class "Gviewer.lvclass">)  [unwired: 8 in]
            n272 = call "SetGraphTime.vi"("error in (no error)"=w658, "Gviewer in"=w659) -> ("error out"=w656:errorcluster, "Gviewer out"=w655:refnum<class "Gviewer.lvclass">)  [unwired: 8 in]
            n273 = call "GV_ToolbarShowTimeSpan.vi"("error in (no error)"=w656, "Gviewer in"=w655) -> ("error out"=w653:errorcluster, "Gviewer out"=w652:refnum<class "Gviewer.lvclass">)  [unwired: 7 in, 1 out]
            n274 = call "GV_StoreNewZoomValue.vi"("Immediate"=w649, "error in (no error)"=w653, "Gviewer in"=w652) -> ("error out"=w650:errorcluster, "Gviewer out"=w651:refnum<class "Gviewer.lvclass">)  [unwired: 7 in]
          }
        }
      }
      event "Graph": Mouse Leave {
        # "Sanity actions when leaving the graph area with mouse"
        n275 = event-data() -> ()  [unwired: 1 in, 1 out]
        n276 = call "GV-MouseUP.vi"("MouseLeave?"=TRUE, "error in (no error)"=w665, "Gviewer in"=w667) -> ("error out"=w666:errorcluster, "Gviewer out"=w668:refnum<class "Gviewer.lvclass">)  [unwired: 7 in]
      }
      event Key Down {
        # "Press a key"
        n277 = event-data() -> ("ScanCode"=w676:i16, "VKey"=w684:T2, "PlatMods.Shift"=w683:bool, "PlatMods.Ctrl"=w682:bool)  [unwired: 1 in]
        n278 = Unbundle By Name(w679) -> ("KeyStrokes_Lookup"=w686:i16[])
        n279 = Get Date/Time In Seconds() -> (seconds since 1Jan1904=w681:timestamp)
        n280 = Search 1D Array(1D array=w686, element=w676) -> (index of element=w680:i32)  [unwired: 1 in]
        n281 = Bundle By Name(cluster=T1 {"Char"=0, "VKey"=enum."ASCII", "Shift"=FALSE, "Ctrl"=FALSE, "Time"=timestamp(0 s since 1904-01-01)} ("Key"), "Char"=w676, "VKey"=w684, "Shift"=w683, "Ctrl"=w682, "Time"=w681) -> (w677:T1)
        n282 = case shown="-1" w680 {
          selector: w680 -> [w693 _]
          tunnel: w679 -> [w687 w707]
          tunnel: w678 -> [w696 w698]
          tunnel: [w696 w699] -> w675
          tunnel: [w688 w700] -> w670
          tunnel: w677 -> [w692 w697]
          tunnel: w676 -> [w691 w704]
          frame Default {
            # "Replace if the switch action already exists"
            n283 = Unbundle By Name(w687) -> ("KeyStrokes_Lookup"=w695:i16[], "KeyStrokes"=w694:T1[])
            n284 = Replace Array Subset(array=w695, new element=w691, index=w693) -> (w690:i16[])
            n285 = Replace Array Subset(array=w694, new element=w692, index=w693) -> (w689:T1[])
            n286 = Bundle By Name(cluster=w687, "KeyStrokes_Lookup"=w690, "KeyStrokes"=w689) -> (w688:refnum<class "Gviewer.lvclass">)
          }
          frame -1 {
            # "Actions on switch pressing\nare in here"
            # "New switch pressure"
            n287 = Unbundle By Name(w707) -> ("KeyStrokes_Lookup"=w706:i16[], "KeyStrokes"=w703:T1[])
            n288 = Build Array (concatenate)(w703, w697) -> (w702:T1[])
            n289 = Build Array (concatenate)(w706, w704) -> (w705:i16[])
            n290 = Bundle By Name(cluster=w707, "KeyStrokes_Lookup"=w705, "KeyStrokes"=w702) -> (w701:refnum<class "Gviewer.lvclass">)
            n291 = call "KeySwitched.vi"("error in (no error)"=w698, "Key"=w697, "Gviewer in"=w701) -> ("error out"=w699:errorcluster, "Gviewer out"=w700:refnum<class "Gviewer.lvclass">)  [unwired: 6 in, 1 out]
            "Key DN" <- w697
          }
        }
        n292 = Unbundle By Name(w670) -> ("GraphCursorLoc"=w669:T20)
        n293 = call "ToolBarButtonDraw.vi"("error in (no error)"=w675, "Gviewer in"=w670) -> ("error out"=w673:errorcluster, "Gviewer out"=w671:refnum<class "Gviewer.lvclass">)  [unwired: 8 in]
        n294 = call "CursorDraw.vi"("error in (no error)"=w673, "Coords"=w669, "Gviewer in"=w671) -> ("error out"=w672:errorcluster, "Gviewer out"=w674:refnum<class "Gviewer.lvclass">)  [unwired: 7 in]
      }
      event Key Up {
        # "Release a key"
        n295 = event-data() -> ("ScanCode"=w715:i16)  [unwired: 1 in]
        n296 = Unbundle By Name(w718) -> ("KeyStrokes_Lookup"=w716:i16[])
        n297 = Search 1D Array(1D array=w716, element=w715) -> (index of element=w719:i32)  [unwired: 1 in]
        n298 = case shown="Default" w719 {
          selector: w719 -> [w728 _]
          tunnel: w718 -> [w729 w735]
          tunnel: w717 -> [w721 w734]
          tunnel: [w726 w735] -> w708
          tunnel: [w722 w734] -> w710
          frame Default {
            w724 = 1 ("index")
            n299 = Unbundle By Name(w729) -> ("KeyStrokes_Lookup"=w733:i16[], "KeyStrokes"=w732:T1[])
            n300 = Delete From Array(array=w733, length=w724, index=w728) -> (array with subset deleted=w731:i16[])  [unwired: 1 out]
            n301 = Delete From Array(array=w732, length=w724, index=w728) -> (deleted portion=w725:T1[], array with subset deleted=w730:T1[])
            n302 = Bundle By Name(cluster=w729, "KeyStrokes_Lookup"=w731, "KeyStrokes"=w730) -> (w727:refnum<class "Gviewer.lvclass">)
            n303 = Index Array(array=w725, index=0) -> (element=w723:T1)
            "Key UP" <- w723
            n304 = call "KeyUnSwitched.vi"("error in (no error)"=w721, "Key"=w723, "Gviewer in"=w727) -> ("error out"=w722:errorcluster, "Gviewer out"=w726:refnum<class "Gviewer.lvclass">)  [unwired: 7 in]
          }
          frame -1 {
          }
        }
        n305 = Unbundle By Name(w708) -> ("GraphCursorLoc"=w713:T20)
        n306 = call "ToolBarButtonDraw.vi"("error in (no error)"=w710, "Gviewer in"=w708) -> ("error out"=w711:errorcluster, "Gviewer out"=w714:refnum<class "Gviewer.lvclass">)  [unwired: 8 in]
        n307 = call "CursorDraw.vi"("error in (no error)"=w711, "Coords"=w713, "Gviewer in"=w714) -> ("error out"=w709:errorcluster, "Gviewer out"=w712:refnum<class "Gviewer.lvclass">)  [unwired: 7 in]
      }
      event Mouse Up {
        # "Detect mouse up event (after dragging action)"
        n308 = event-data() -> ("Coords"=w737:T20)  [unwired: 1 in]
        n309 = call "GV-MouseUP.vi"("MouseLeave?"=FALSE, "error in (no error)"=w738, "Coords"=w737, "Gviewer in"=w740) -> ("error out"=w739:errorcluster, "Gviewer out"=w741:refnum<class "Gviewer.lvclass">)  [unwired: 6 in]
      }
      event "ToolBar": Mouse Move {
        # "Update toolbar icons when hovering over it"
        n310 = event-data() -> ("Coords"=w746:T20)  [unwired: 1 in]
        n311 = call "ToolBarButtonDraw.vi"("error in (no error)"=w747, "Coords"=w746, "Gviewer in"=w748) -> ("error out"=w743:errorcluster, "Gviewer out"=w745:refnum<class "Gviewer.lvclass">)  [unwired: 7 in]
        n312 = call "GV_ToolbarShowTimeSpan.vi"("error in (no error)"=w743, "Gviewer in"=w745) -> ("error out"=w742:errorcluster, "Gviewer out"=w744:refnum<class "Gviewer.lvclass">)  [unwired: 7 in, 1 out]
      }
      event "ToolBar": Mouse Down {
        # "Press a button on the toolbar"
        n313 = event-data() -> ("Coords"=w749:T20)  [unwired: 1 in]
        n314 = Unbundle By Name(w757) -> ("ToolButtonFocus"=w754:i32)
        n315 = Bundle By Name(cluster=w757, "ToolButtonSelected"=w754) -> (w756:refnum<class "Gviewer.lvclass">)
        n316 = call "ToolBarButtonDraw.vi"("error in (no error)"=w755, "Coords"=w749, "Gviewer in"=w756) -> ("error out"=w753:errorcluster, "Gviewer out"=w751:refnum<class "Gviewer.lvclass">)  [unwired: 7 in]
        n317 = case shown="Default" w754 {
          tunnel: w753 -> [w759 w763 w777]
          tunnel: [w759 w762 w775] -> w752
          tunnel: w751 -> [w758 w761 w778]
          tunnel: [w758 w760 w776] -> w750
          tunnel: w749 -> [_ _ w774]
          frame Default {
          }
          frame 0 {
            w764 = -1  # Remove Selection
            # "Escape"
            n318 = Unbundle By Name(w761) -> ("TagSelection"=w765:string[], "Graph-ref"=w766:refnum<vi>)
            n319 = for {
              tunnel: w766 -> [w773]
              shift-right: [w769] -> w762
              shift-left: w763 -> [w771]
              tunnel: w765 -> [_] mode=indexing
              i -> [w768]
              # "Remove any trace selection"
              n320 = property class="XYGraph (strict)"(reference=w773, error in=w771, "Active Plot"=w768) -> (reference out=w772:refnum<vi>, error out=w770:errorcluster)
              n321 = property class="XYGraph (strict)"(reference=w772, error in=w770, "Plot.Line Width"=u8 1) -> (error out=w769:errorcluster)  [unwired: 1 out]
            }
            n322 = Bundle By Name(cluster=w761, "PlotSelected"=w764) -> (w760:refnum<class "Gviewer.lvclass">)
          }
          frame 1 {
            # "Undo"
            n323 = call "GV_undo.vi"("error in (no error)"=w777, "Coords"=w774, "Gviewer in"=w778) -> ("error out"=w775:errorcluster, "Gviewer out"=w776:refnum<class "Gviewer.lvclass">)  [unwired: 7 in]
          }
        }
      }
      event Value Change {
        # "Set Graph mode to 'live' (continous updates)"
        n324 = event-data() -> ("NewVal"=w783:T3)  [unwired: 1 in]
        n325 = Bundle By Name(cluster=w788, "Live"=w783) -> (w782:refnum<class "Gviewer.lvclass">)
        n326 = call "Request_Gserver_Update.vi"("error in (no error)"=w779, "Gviewer in"=w782) -> ("error out"=w784:errorcluster, "Gviewer out"=w785:refnum<class "Gviewer.lvclass">)  [unwired: 8 in]
        n327 = call "SetGraphTime.vi"("error in (no error)"=w784, "Gviewer in"=w785) -> ("error out"=w786:errorcluster, "Gviewer out"=w787:refnum<class "Gviewer.lvclass">)  [unwired: 8 in]
        n328 = call "GV_DrawLiveBox.vi"("error in (no error)"=w786, "Gviewer in"=w787) -> ("error out"=w780:errorcluster, "Gviewer out"=w781:refnum<class "Gviewer.lvclass">)  [unwired: 8 in]
      }
      event Panel Close? {
        # "On closing action of this Graph: Ask the Gserver to perform the closing (to ensure that reference in Gserver is removed)"
        n329 = event-data() -> ()  [unwired: 1 in, 4 out]
        n330 = call "SendDataToServer.vi"("Query_type"=Typedef_QueryType."CloseClient", "Gviewer in"=w792) -> ("Gviewer out"=w791:refnum<class "Gviewer.lvclass">)  [unwired: 8 in, 1 out]
        n331 = event-data("Discard?"=TRUE) -> ()  [unwired: 1 in, 1 out]
      }
    }
  }
  n332 = call "GV_Destructor.vi"("error in (no error)"=w10, "Gviewer in"=w1) -> ()  [unwired: 8 in, 2 out]
